vi "Merge Four Arrays for SDL Write 1D Double.vi"(8 "array 4 in":dbl[](array[numeric]), 9 "array 3 in":dbl[](array[numeric]), 10 "array 2 in":dbl[](array[numeric]), 11 "array 1 in":dbl[](array[numeric])) -> (3 "array out":dbl[](array[numeric]))   [LabVIEW 2026]
doc: "Merges four 1D DBL arrays into one 1D DBL array for FlexLogger SDL Write 1D Double."
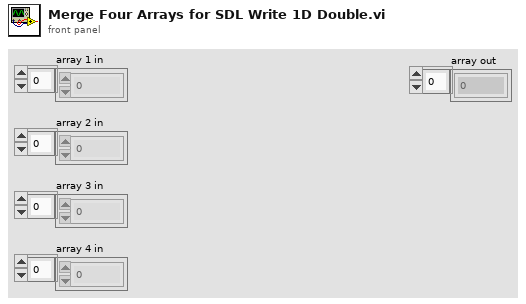
[diagram p1: front panel]
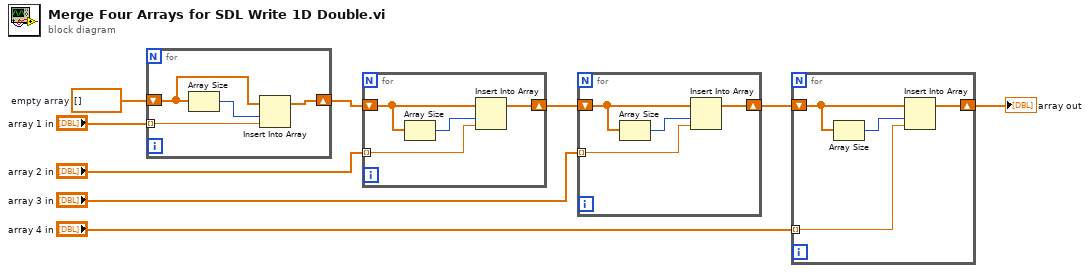
[diagram p0: block diagram]
diagram:
  w8 = dbl[] []  # empty array
  n1 = for {
    tunnel: "array 1 in" -> [w12] mode=indexing
    shift-right: [w11] -> w6
    shift-left: w8 -> [w10]
    n2 = Array Size(array=w10) -> (size(s)=w13:i32)
    n3 = Insert Into Array(array=w10, index=w13, new element=w12) -> (w11:dbl[])
  }
  n4 = for {
    tunnel: "array 2 in" -> [w16] mode=indexing
    shift-right: [w15] -> w4
    shift-left: w6 -> [w14]
    n5 = Array Size(array=w14) -> (size(s)=w17:i32)
    n6 = Insert Into Array(array=w14, index=w17, new element=w16) -> (w15:dbl[])
  }
  n7 = for {
    tunnel: "array 3 in" -> [w20] mode=indexing
    shift-right: [w19] -> w2
    shift-left: w4 -> [w18]
    n8 = Array Size(array=w18) -> (size(s)=w21:i32)
    n9 = Insert Into Array(array=w18, index=w21, new element=w20) -> (w19:dbl[])
  }
  n10 = for {
    tunnel: "array 4 in" -> [w24] mode=indexing
    shift-right: [w23] -> w1
    shift-left: w2 -> [w22]
    n11 = Array Size(array=w22) -> (size(s)=w25:i32)
    n12 = Insert Into Array(array=w22, index=w25, new element=w24) -> (w23:dbl[])
  }
  "array out" <- w1
